vi "Helper Loop Map FGV.vi"(6 "Action":T2, 10 "Helper Loop VI Reference In":refnum<vi>, 11 "Helper Loop In":refnum<class "Helper Loop.lvclass">) -> (1 "Get Helper Loop":bool, 2 "Helper Loop VI Reference Out":refnum<vi>, 3 "Helper Loop Out":refnum<class "Helper Loop.lvclass">, 5 "All Helper Queues":T1(array[cluster]))   [LabVIEW 2026, in "Helper Loop.lvclass"]
doc: "ヘルパーループのクラスと呼び出したVIリファレンスのMapを取り扱うFGVです。"
uses:
  Helper Loop.lvclass
  Helper Loop Map FGV Action.ctl
  Helper Loop Map.ctl
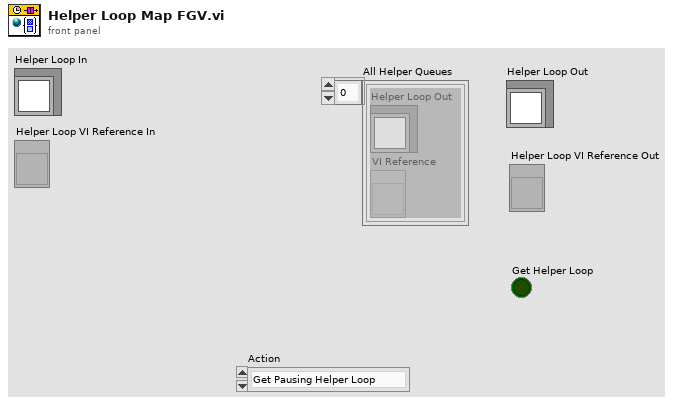
[diagram p1: front panel]
types:
  T1 = cluster{"Helper Loop Out":refnum<class "Helper Loop.lvclass">, "VI Reference":refnum<vi>}[]
  T2 = typedef "Helper Loop.lvclass/Helper Loop Map FGV Action.ctl" = enum16{"Get Pausing Helper Loop", "Register Active Helper Loop", "Pause Helper Loop", "Close Helper Loop", "Get All Helper Loops"}
  T3 = typedef "Helper Loop.lvclass/Helper Loop Map.ctl" = map{refnum<class "Helper Loop.lvclass">, refnum<vi>}
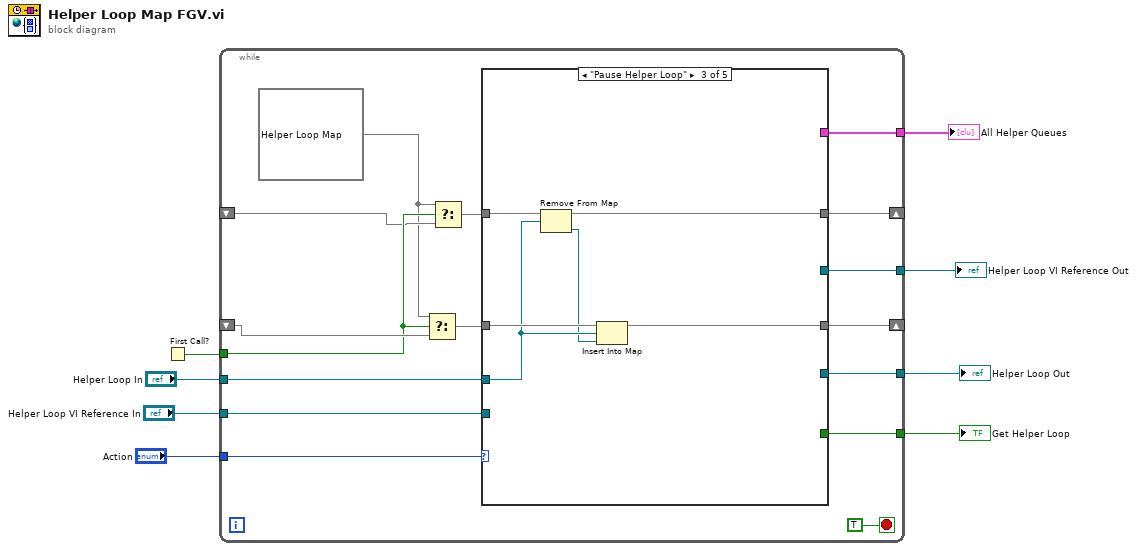
[diagram p0: block diagram]
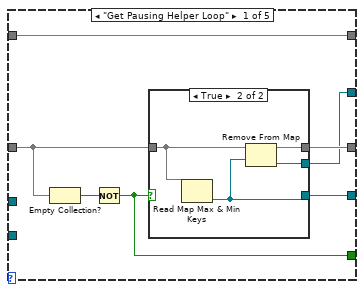
[diagram p2: hidden frame]
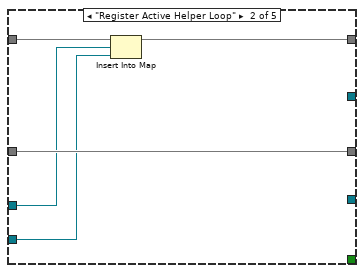
[diagram p4: hidden frame]
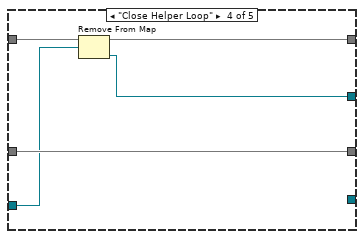
[diagram p5: hidden frame]
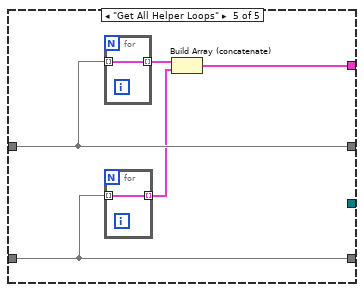
[diagram p6: hidden frame]
diagram:
  n1 = First Call?() -> (First Call?: T/F=w7:bool)
  n2 = while {
    tunnel: "Action" -> [w23]
    tunnel: w7 -> [w19]
    shift-right: [w22] -> _
    shift-left: _ -> [w16]
    shift-right: [w21] -> _
    shift-left: _ -> [w20]
    tunnel: [w15] -> w6
    tunnel: [w14] -> w5
    tunnel: "Helper Loop In" -> [w13]
    tunnel: [w12] -> w1
    tunnel: "Helper Loop VI Reference In" -> [w10]
    tunnel: [w9] -> w2
    stop <- TRUE stop-if-true
    w11 = T3 {} ("Helper Loop Map In")
    n3 = Select(t=w11, s=w19, f=w20) -> (s? t:f=w17:T3)
    n4 = Select(t=w11, s=w19, f=w16) -> (s? t:f=w18:T3)
    n5 = case shown="\"Pause Helper Loop\"" w23 {
      tunnel: [w31 w39 w43 w49 w57] -> w22
      tunnel: [w28 w41 w46 w52 w56] -> w21
      tunnel: w18 -> [w31 w40 w45 w51 w57]
      tunnel: w17 -> [w30 w41 w47 w52 w56]
      tunnel: [w25 _ _ _ _] -> w15
      tunnel: [w29 _ _ _ _] -> w14
      tunnel: w13 -> [_ w38 w44 w50 _]
      tunnel: [_ _ _ _ w53] -> w12
      tunnel: w10 -> [_ w37 _ _ _]
      tunnel: [w27 _ _ w48 _] -> w9
      frame "Get Pausing Helper Loop" {
        n6 = Empty Collection?(1:w30) -> (0:w26:bool)
        n7 = Not(x=w26) -> (.not. x?=w25:bool)
        n8 = case shown="True" w25 {
          tunnel: w30 -> [w32 w36]
          tunnel: [_ w35] -> w29
          tunnel: [w32 w34] -> w28
          tunnel: [_ w33] -> w27
          frame False {
          }
          frame True {
            n9 = Read Map Max & Min Keys(11:w36) -> (1:w35:refnum<class "Helper Loop.lvclass">)  [unwired: 1 out]
            n10 = Remove From Map(10:w35, 11:w36) -> (1:w33:refnum<vi>, 3:w34:T3)  [unwired: 1 out]
          }
        }
      }
      frame "Register Active Helper Loop" {
        n11 = Insert Into Map(map in=w40, key=w38, value=w37) -> (map out=w39:T3)  [unwired: 2 out]
      }
      frame "Pause Helper Loop" {
        n12 = Remove From Map(10:w44, 11:w45) -> (1:w42:refnum<vi>, 3:w43:T3)  [unwired: 1 out]
        n13 = Insert Into Map(map in=w47, key=w44, value=w42) -> (map out=w46:T3)  [unwired: 2 out]
      }
      frame "Close Helper Loop" {
        n14 = Remove From Map(10:w50, 11:w51) -> (1:w48:refnum<vi>, 3:w49:T3)  [unwired: 1 out]
      }
      frame "Get All Helper Loops" {
        n15 = for {
          tunnel: [w59] -> w55 mode=indexing
          tunnel: w57 -> [w59] mode=indexing
        }
        n16 = for {
          tunnel: [w58] -> w54 mode=indexing
          tunnel: w56 -> [w58] mode=indexing
        }
        n17 = Build Array (concatenate)(w55, w54) -> (w53:T1)
      }
    }
  }
  "Get Helper Loop" <- w6
  "Helper Loop Out" <- w5
  "Helper Loop VI Reference Out" <- w2
  "All Helper Queues" <- w1
